vi "Register Execution.vi"(0 "Engine  In":T1, 7 "Execution":T2, 11 "error in (no error)":errorcluster) -> (4 "Engine":T1, 15 "error out":errorcluster)   [LabVIEW 2020, in "TSS.lvlib" / "Engine.lvclass"]
uses:
  Engine.lvclass
  Execution/Typedefs/Session Handle.ctl
  Execution/Execution.lvclass
  Typedefs/Session Handle.ctl
  Engine.lvclass/Engine.ctl
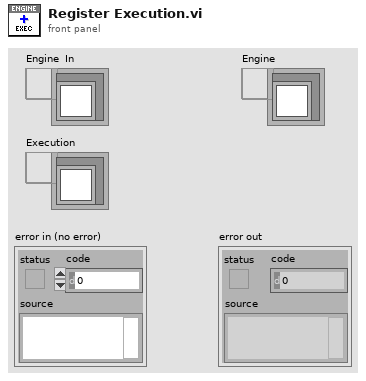
[diagram p1: front panel]
types:
  T1 = typedef "TSS.lvlib/Engine.lvclass/Session Handle.ctl" = refnum<data-value>
  T2 = typedef "TSS.lvlib/Execution.lvclass/Session Handle.ctl" = refnum<data-value>
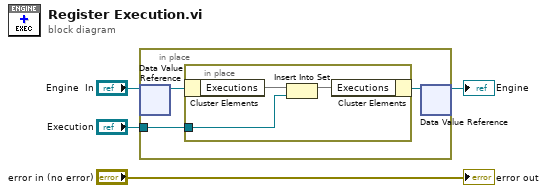
[diagram p0: block diagram]
diagram:
  n1 = in-place {
    in-place-border: "Execution" -> [w7]
    n2 = in-place-dvr #1("Engine  In") -> (w6:refnum<class "Engine.lvclass">)  [unwired: 1 out]
    n3 = in-place {
      in-place-border: w7 -> [w9]
      n4 = in-place-cluster #2(w6) -> ("Executions"=w10:set{T2})
      n5 = Insert Into Set(10:w9, 11:w10) -> (3:w8:set{T2})  [unwired: 1 out]
      n6 = in-place-cluster #2("Executions"=w8) -> (w5:refnum<class "Engine.lvclass">)
    }
    n7 = in-place-dvr #1(w5) -> (→"Engine":T1)  [unwired: 1 out]
  }
  "error out" <- "error in (no error)"
